vi "Build CE Deploy - Update CLFN.vi"(8 "error in":errorcluster, 11 "Project":refnum<vi>) -> (0 "error out":errorcluster, 3 "dup Project":refnum<vi>)   [LabVIEW 2021]
doc: "::: CalcExpress Toolkit :::\nCopyright (c) 2000-2026 Konstantin Shifershteyn. All rights reserved."
uses:
  <vilib>/Utility/traverseref.llb/TRef TravTarget.ctl
  <vilib>/Utility/traverseref.llb/VI Scripting - Traverse.lvlib
panel:
  out "Updated VIs":path[](array[path])
  # "CalcExpress Toolkit\nCopyright (c) 2000-2026 Konstantin Shifershteyn"
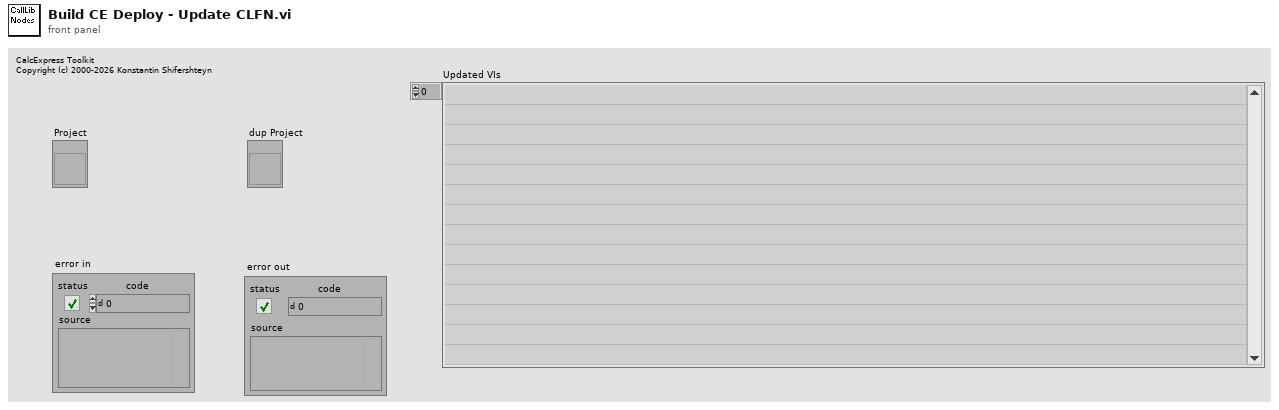
[diagram p1: front panel]
types:
  T1 = typedef "TRef TravTarget.ctl" = enum16{"FP", "BD", "Other"}
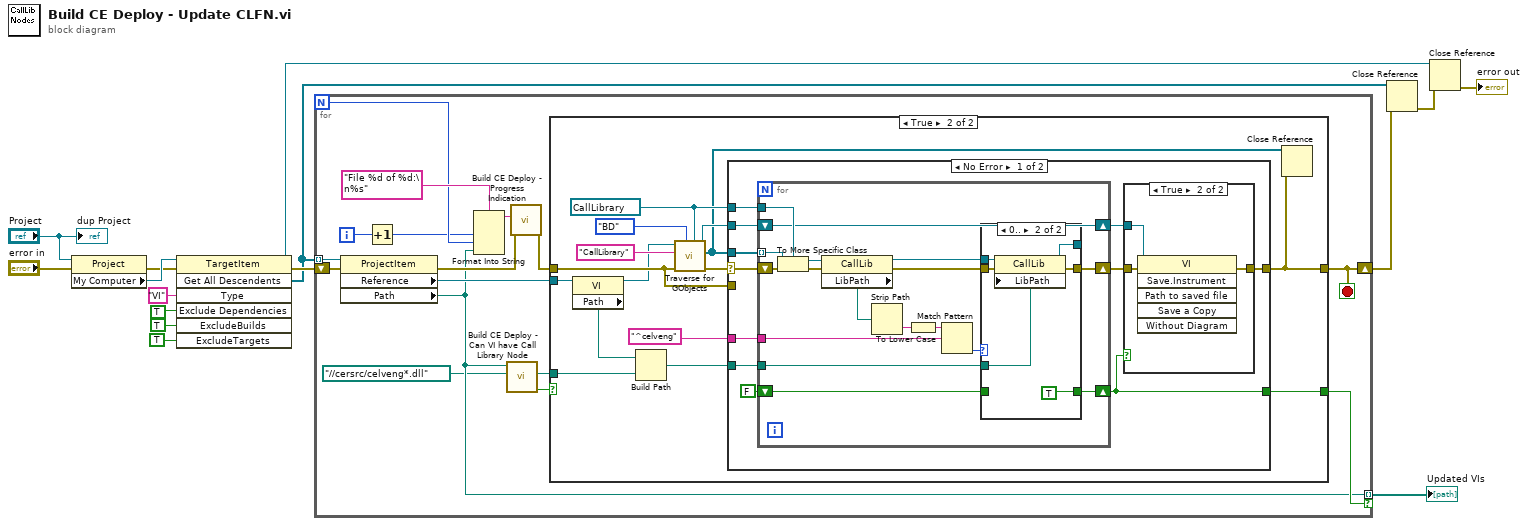
[diagram p0: block diagram]
diagram:
  n1 = property class="Project"(reference="Project", error in="error in") -> (error out=w11:errorcluster, "My Computer"=w15:refnum<vi>)  [unwired: 1 out]
  n2 = invoke class="TargetItem" method="Get All Descendents"(reference=w15, error in=w11, "Type"="VI", "Exclude Dependencies"=TRUE, "ExcludeBuilds"=TRUE, "ExcludeTargets"=TRUE) -> (reference out=w9:refnum<vi>, error out=w10:errorcluster, "All Descendents"=w4:refnum<vi>[])  [unwired: 1 in, 4 out]
  n3 = for {
    N -> [w22]
    tunnel: w4 -> [w31] mode=indexing
    shift-right: [w25] -> w3
    shift-left: w10 -> [w30]
    tunnel: [w18] -> w8 mode=indexing if=w29
    i -> [w23]
    stop <- w25 stop-if-true
    n4 = property class="ProjectItem"(reference=w31, error in=w30) -> (error out=w20:errorcluster, "Reference"=w26:refnum<vi>, "Path"=w18:path)  [unwired: 1 out]
    n5 = Increment(x=w23) -> (x+1=w21:i32)
    n6 = Format Into String(format string="File %d of %d:\n%s", w21, w22, w18) -> (resulting string=w17:string)  [unwired: 2 in, 1 out]
    n7 = call "Build CE Deploy - Can VI have Call Library Node.vi"("default relative path to DLL"=path "../../cersrc/celveng*.dll", "VI Path"=w18) -> ("Can have CLN"=w28:bool, "celveng*.dll path relative to VI"=w27:path)  [unwired: 8 in]
    n8 = call "Build CE Deploy - Progress Indication.vi"("error in"=w20, "message 2"=w17) -> ("error out"=w19:errorcluster)  [unwired: 9 in]
    n9 = case shown="True" w28 {
      tunnel: [w32 w35] -> w25
      tunnel: w26 -> [_ w38]
      tunnel: w19 -> [w32 w39]
      tunnel: [_ w41] -> w29
      tunnel: w27 -> [_ w34]
      frame False {
      }
      frame True {
        w47 = refnum<vi> refnum ("Other Refnum")
        n10 = property class="VI"(reference=w38) -> (reference out=w36:refnum<vi>, "Path"=w37:path)  [unwired: 1 in, 1 out]
        n11 = Build Path(base path=w37, name or relative path=w34) -> (appended path=w33:path)
        n12 = call <vilib>:"Traverse for GObjects.vi"("Other Refnum"=w47, "Traverse Target"=TRef_TravTarget."BD", "error in (no error)"=w39, "Class Name"="CallLibrary", "VI Refnum"=w36) -> ("error out"=w40:errorcluster, "References"=w44:refnum<vi>[], "dup VI Refnum"=w46:refnum<vi>)  [unwired: 3 in, 1 out]
        n13 = case shown="No Error" w40 {
          selector: w40 -> [w53 _]
          tunnel: w33 -> [w58 _]
          tunnel: w47 -> [w57 _]
          tunnel: w46 -> [w55 _]
          tunnel: "^celveng" -> [w54 _]
          tunnel: w44 -> [w49 _]
          tunnel: [w48 w89] -> w35
          tunnel: [w50 _] -> w41
          tunnel: w39 -> [_ w89]
          frame No Error {
            n14 = for {
              shift-right: [w63] -> w51
              shift-left: w53 -> [w79]
              tunnel: w49 -> [w78] mode=indexing
              tunnel: w57 -> [w77]
              tunnel: w54 -> [w72]
              shift-right: [w67] -> w52
              shift-left: w55 -> [w67]
              shift-right: [w66] -> w50
              shift-left: FALSE -> [w65]
              tunnel: w58 -> [w64]
              n15 = To More Specific Class(target class=w77, reference=w78, error in=w79) -> (specific class reference=w75:refnum<vi>, error out=w76:errorcluster)
              n16 = property class="CallLib"(reference=w75, error in=w76) -> (reference out=w68:refnum<vi>, error out=w69:errorcluster, "LibPath"=w74:path)
              n17 = Strip Path(path=w74) -> (name=w73:string)  [unwired: 1 out]
              n18 = To Lower Case(string=w73) -> (all lower case string=w71:string)
              n19 = Match Pattern(string=w71, regular expression=w72) -> (offset past match=w70:i32)  [unwired: 1 in, 3 out]
              n20 = case shown="0.." w70 {
                tunnel: [w82 w86] -> w63
                tunnel: w69 -> [w82 w88]
                tunnel: w68 -> [w81 w87]
                tunnel: [w81 w85] -> _
                tunnel: [w80 TRUE] -> w66
                tunnel: w65 -> [w80 _]
                tunnel: w64 -> [_ w83]
                frame ..-1 {
                }
                frame 0.. {
                  n21 = property class="CallLib"(reference=w87, error in=w88, "LibPath"=w83) -> (reference out=w85:refnum<vi>, error out=w86:errorcluster)
                }
              }
            }
            n22 = case shown="True" w50 {
              tunnel: w52 -> [_ w62]
              tunnel: w51 -> [w59 w61]
              tunnel: [w59 w60] -> w48
              frame False {
              }
              frame True {
                n23 = invoke class="VI" method="Save.Instrument"(reference=w62, error in=w61) -> (error out=w60:errorcluster)  [unwired: 4 in, 5 out]
              }
            }
          }
          frame Error {
          }
        }
        n24 = Close Reference(reference=w44, error in (no error)=w35) -> ()  [unwired: 1 out]
      }
    }
  }
  "Updated VIs" <- w8
  n25 = Close Reference(reference=w4, error in (no error)=w3) -> (error out=w2:errorcluster)
  n26 = Close Reference(reference=w9, error in (no error)=w2) -> (error out=→"error out":errorcluster)
  "dup Project" <- "Project"
